vi "SeqEditor_ParamINput.vi"(8 "error in (no error)":errorcluster, 11 "NLTest in":refnum<class "NLTest.lvclass">) -> (0 "error out":errorcluster, 3 "NLTest out":refnum<class "NLTest.lvclass">)   [LabVIEW 2017, in "NLTest.lvclass"]
uses:
  NLTest.lvclass
  NLTest.lvclass/NLTest.ctl
  <vilib>/Utility/miscctls.llb/LVRowAndColumnTypeDef.ctl
  <vilib>/Utility/miscctls.llb/LVSelectionTypeDef.ctl
  SeqEditor_Global.vi
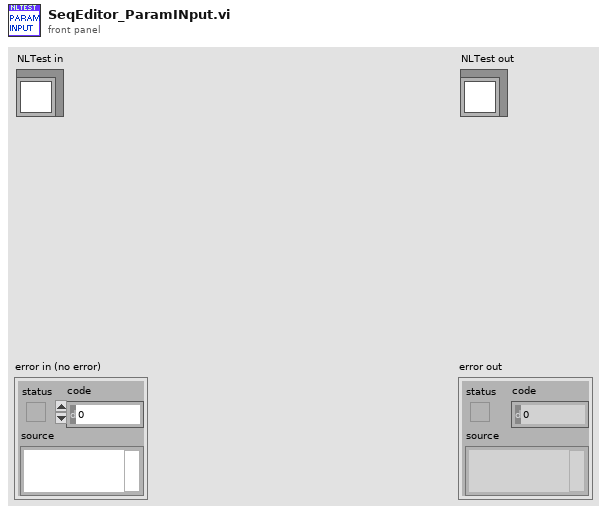
[diagram p1: front panel]
types:
  T1 = typedef "LVRowAndColumnTypeDef.ctl" = cluster{"Row":i32, "Column":i32}
  T2 = typedef "LVSelectionTypeDef.ctl" = cluster{"Selection Start":u32, "Selection End":u32}
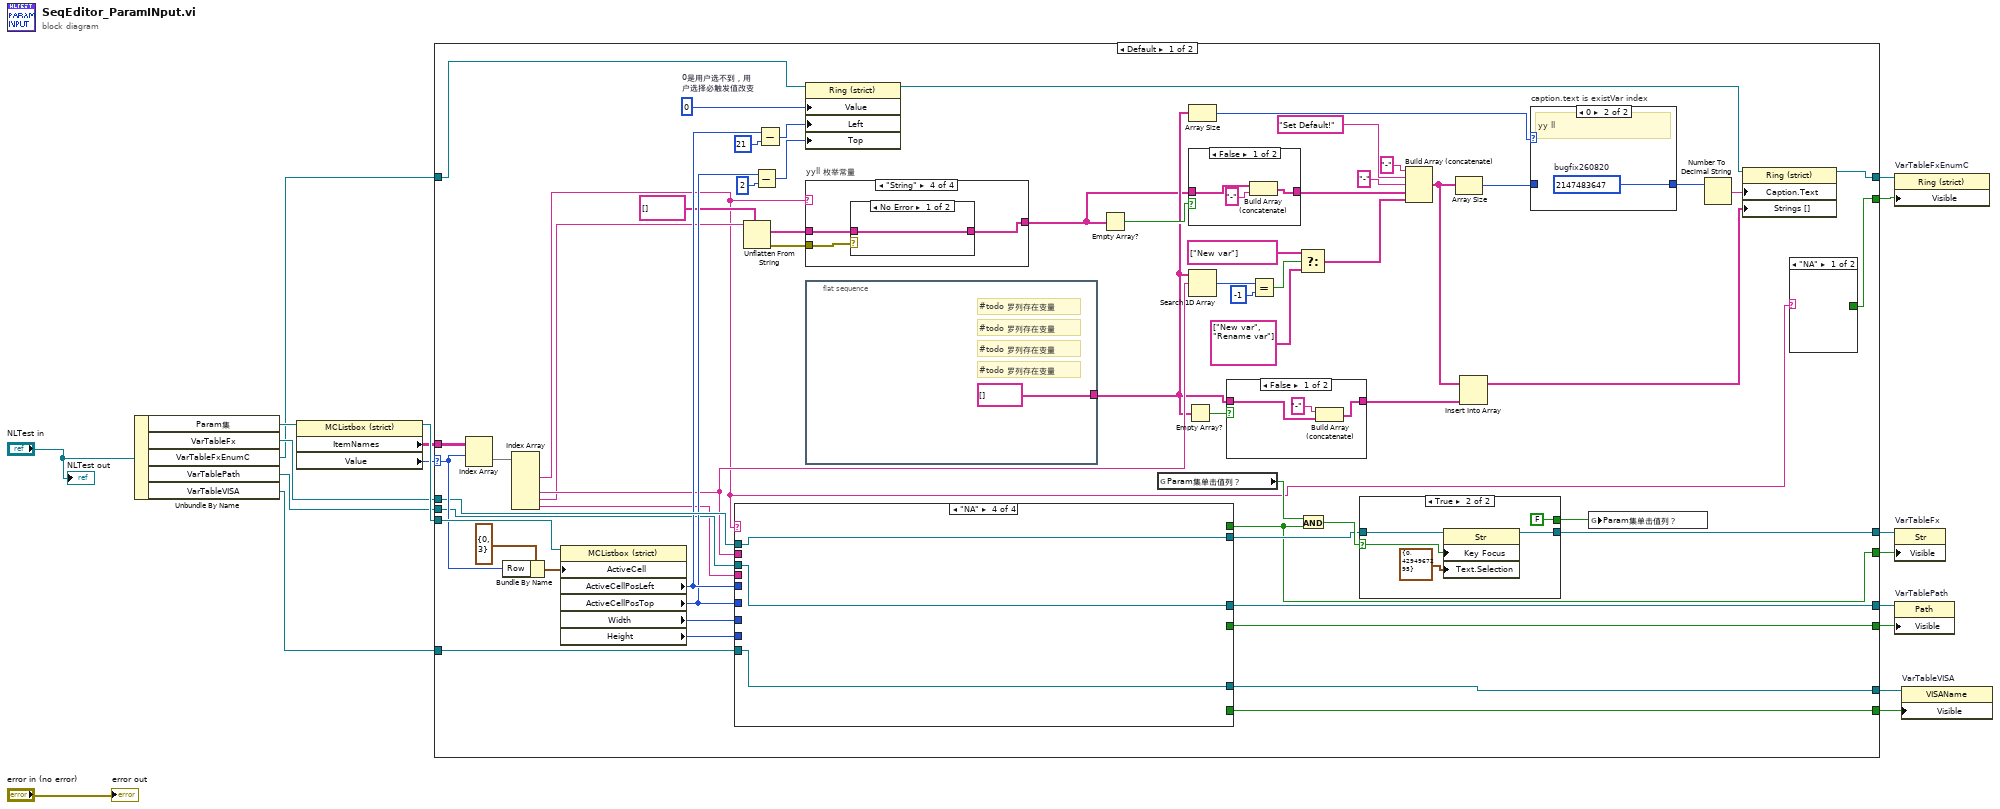
[diagram p0: block diagram]
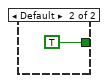
[diagram p2: hidden frame]
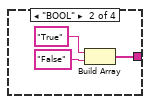
[diagram p4: hidden frame]
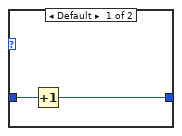
[diagram p7: hidden frame]
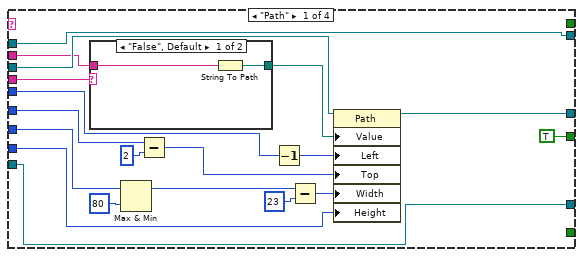
[diagram p11: hidden frame]
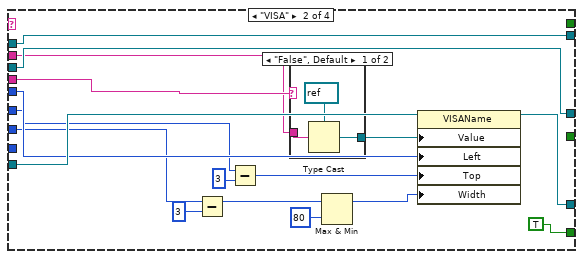
[diagram p13: hidden frame]
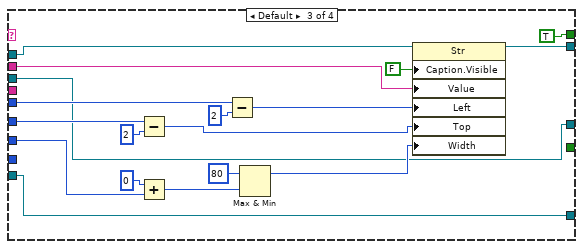
[diagram p15: hidden frame]
diagram:
  n1 = Unbundle By Name("NLTest in") -> ("Param集"=w16:refnum<vi>, "VarTableFx"=w12:refnum<vi>, "VarTableFxEnumC"=w9:refnum<vi>, "VarTablePath"=w5:refnum<vi>, "VarTableVISA"=w1:refnum<vi>)
  n2 = property on="Property Node" class="MCListbox (strict)"(reference=w16) -> (reference out=w15:refnum<vi>, "ItemNames"=w14:string[][], "Value"=w13:i32)  [unwired: 1 in, 1 out]
  n3 = case shown="Default" w13 {
    selector: w13 -> [w74 _]
    tunnel: w15 -> [w78 _]
    tunnel: w14 -> [w77 _]
    tunnel: w12 -> [w72 w170]
    tunnel: [w58 w170] -> w11
    tunnel: [w28 _] -> w10
    tunnel: w9 -> [w68 w171]
    tunnel: [w39 w171] -> w8
    tunnel: [w27 _] -> w7
    tunnel: [w26 _] -> w6
    tunnel: w5 -> [w25 w169]
    tunnel: [w24 w169] -> w4
    tunnel: w1 -> [w22 w168]
    tunnel: [w21 w168] -> w3
    tunnel: [w20 _] -> w2
    frame Default {
      w69 = u16 0  # 0是用户选不到，用 户选择必触发值改变
      n4 = Index Array(array=w77, index (row)=w74) -> (element=w76:string[])  [unwired: 1 in]
      n5 = Bundle By Name(cluster=T1 {"Row"=0, "Column"=3} ("Active Cell:Active Cell"), "Row"=w74) -> (w75:T1)
      n6 = Index Array(array=w76) -> (element #2=w19:string, element #4=w35:string, element #5=w29:string, element #6=w23:string)  [unwired: 6 in, 2 out]
      n7 = property class="MCListbox (strict)"(reference=w78, "ActiveCell"=w75) -> ("ActiveCellPosLeft"=w63:i32, "ActiveCellPosTop"=w62:i32, "Width"=w71:u32, "Height"=w70:u32)  [unwired: 1 in, 2 out]
      n8 = case shown="\"NA\"" w19 {
        tunnel: w72 -> [w124 w134 w157 w167]
        tunnel: w35 -> [w112 w132 w156 _]
        tunnel: w63 -> [w110 w131 w155 _]
        tunnel: w62 -> [w109 w130 w154 _]
        tunnel: w71 -> [w108 w129 w153 _]
        tunnel: w70 -> [w107 _ _ _]
        tunnel: [w124 w134 w151 w167] -> w59
        tunnel: [_ _ TRUE _] -> w27
        tunnel: [TRUE _ _ _] -> w26
        tunnel: w25 -> [w114 w135 w148 w166]
        tunnel: [w113 w135 w148 w166] -> w24
        tunnel: w23 -> [w111 w133 _ _]
        tunnel: w22 -> [w106 w138 w147 w165]
        tunnel: [w106 w137 w147 w165] -> w21
        tunnel: [_ TRUE _ _] -> w20
        frame "Path" {
          n9 = case shown="\"False\", Default" w111 {
            tunnel: w112 -> [w126 _]
            tunnel: [w125 _] -> w122
            frame "False", Default {
              n10 = String To Path(string=w126) -> (path=w125:path)
            }
            frame "True" {
            }
          }
          n11 = Max & Min(x=w108, y=u32 80) -> (max(x,y)=w118:u32)  [unwired: 1 out]
          n12 = Subtract(x=w109, y=2) -> (x-y=w116:i32)
          n13 = Decrement(x=w110) -> (x-1=w117:i32)
          n14 = Subtract(x=w118, y=u32 23) -> (x-y=w121:u32)
          n15 = property class="Path"(reference=w114, "Value"=w122, "Left"=w117, "Top"=w116, "Width"=w121, "Height"=w107) -> (reference out=w113:refnum<vi>)  [unwired: 1 in, 1 out]
        }
        frame "VISA" {
          n16 = Subtract(x=w129, y=u32 3) -> (x-y=w128:u32)
          n17 = Subtract(x=w130, y=3 ("x")) -> (x-y=w140:i32)
          n18 = case shown="\"False\", Default" w133 {
            tunnel: w132 -> [w145 _]
            tunnel: [w144 _] -> w143
            frame "False", Default {
              n19 = Type Cast(type=refnum<visa-resource-name> refnum ("Value"), x=w145) -> (*(type *) &x=w144:refnum<visa-resource-name>)
            }
            frame "True" {
            }
          }
          n20 = Max & Min(x=w128, y=u32 80) -> (max(x,y)=w141:u32)  [unwired: 1 out]
          n21 = property class="VISAName"(reference=w138, "Value"=w143, "Left"=w131, "Top"=w140, "Width"=w141) -> (reference out=w137:refnum<vi>)  [unwired: 1 in, 1 out]
        }
        frame Default {
          n22 = Subtract(x=w154, y=2) -> (x-y=w158:i32)
          n23 = Add(x=u32 0, y=w153) -> (x+y=w162:u32)
          n24 = Subtract(x=w155, y=2 ("x")) -> (x-y=w159:i32)
          n25 = Max & Min(x=u32 80, y=w162) -> (max(x,y)=w161:u32)  [unwired: 1 out]
          n26 = property class="Str"(reference=w157, "Caption.Visible"=FALSE, "Value"=w156, "Left"=w159, "Top"=w158, "Width"=w161) -> (reference out=w151:refnum<vi>)  [unwired: 1 in, 1 out]
        }
        frame "NA" {
        }
      }
      n27 = Unflatten From String(type=string[] [], binary string=w29) -> (value=w32:string[], error out=w31:errorcluster)  [unwired: 3 in, 1 out]
      n28 = Subtract(x=w62, y=2) -> (x-y=w64:i32)
      n29 = Subtract(x=w63, y=21) -> (x-y=w65:i32)
      n30 = property class="Ring (strict)"(reference=w68, "Value"=w69, "Left"=w65, "Top"=w64) -> (reference out=w40:refnum<vi>)  [unwired: 1 in, 1 out]
      n31 = case "yyll 枚举常量" shown="\"String\"" w19 {
        tunnel: w32 -> [w80 _ _ w84]
        tunnel: [w80 w81 _ w85] -> w30
        tunnel: w31 -> [_ _ _ w86]
        frame Default {
        }
        frame "BOOL" {
          n32 = Build Array("True" ("y"), "False" ("y")) -> (w81:string[])
        }
        frame "Number" {
        }
        frame "String" {
          n33 = case shown="No Error" w86 {
            tunnel: [w87 _] -> w85
            tunnel: w84 -> [w87 _]
            frame No Error {
            }
            frame Error {
            }
          }
        }
      }
      n34 = flat-sequence {
        tunnel: [string[] [] ("1D array")] -> w34
        frame #0 {
          # "#todo 罗列存在变量"
          # "#todo 罗列存在变量"
          # "#todo 罗列存在变量"
          # "#todo 罗列存在变量"
        }
      }
      n35 = Empty Array?(array=w30) -> (empty?=w56:bool)
      n36 = global read "SeqEditor_Global.vi" "Param集单击值列？"() -> (w60:bool)
      n37 = Empty Array?(array=w34) -> (empty?=w54:bool)
      n38 = Array Size(array=w34) -> (size(s)=w52:i32)
      n39 = case shown="False" w56 {
        tunnel: [w97 w99] -> w55
        tunnel: w30 -> [w98 w99]
        frame False {
          n40 = Build Array (concatenate)(w98, "-" ("element")) -> (w97:string[])
        }
        frame True {
        }
      }
      n41 = Search 1D Array(1D array=w34, element=w35) -> (index of element=w38:i32)  [unwired: 1 in]
      n42 = case shown="False" w54 {
        tunnel: [w93 w95] -> w53
        tunnel: w34 -> [w94 w95]
        frame False {
          n43 = Build Array (concatenate)("-" ("element"), w94) -> (w93:string[])
        }
        frame True {
        }
      }
      n44 = Equal?(x=w38, y=-1) -> (x = y?=w36:bool)
      n45 = Select(t=string[] ["New var"], s=w36, f=string[] ["New var", "Rename var"]) -> (s? t:f=w44:string[])
      n46 = And(x=w60, y=w27) -> (x .and. y?=w61:bool)
      n47 = case shown="True" w61 {
        selector: w61 -> [_ w103]
        tunnel: [_ FALSE ("Parmcol2hit")] -> w57
        tunnel: w59 -> [w100 w104]
        tunnel: [w100 w101] -> w58
        frame False {
        }
        frame True {
          n48 = property class="Str"(reference=w104, "Key Focus"=w103, "Text.Selection"=T2 {"Selection Start"=0, "Selection End"=4294967295}) -> (reference out=w101:refnum<vi>)  [unwired: 1 in, 1 out]
        }
      }
      n49 = Build Array (concatenate)("-" ("element"), "Set Default!" ("String"), "-" ("element"), w55, w44) -> (w50:string[])
      n50 = Array Size(array=w50) -> (size(s)=w49:i32)
      n51 = Insert Into Array(array=w50, new element=w53) -> (w47:string[])  [unwired: 1 in]
      n52 = case "caption.text is existVar index" shown="0" w52 {
        tunnel: [w89 w91] -> w51
        tunnel: w49 -> [w90 _]
        frame Default {
          n53 = Increment(x=w90) -> (x+1=w89:i32)
        }
        frame 0 {
          w91 = 2147483647  # bugfix260820
          # "yy ll"
        }
      }
      n54 = global write "SeqEditor_Global.vi" "Param集单击值列？"(w57) -> ()
      n55 = Number To Decimal String(number=w51) -> (decimal integer string=w46:string)  [unwired: 1 in]
      n56 = property class="Ring (strict)"(reference=w40, "Caption.Text"=w46, "Strings []"=w47) -> (reference out=w39:refnum<vi>)  [unwired: 1 in, 1 out]
      n57 = case shown="\"NA\"" w19 {
        tunnel: [_ TRUE] -> w28
        frame "NA" {
        }
        frame Default {
        }
      }
    }
    frame ..-1 {
    }
  }
  n58 = property on="VarTableFxEnumC" class="Ring (strict)"(reference=w8, "Visible"=w10) -> ()  [unwired: 1 in, 2 out]
  n59 = property on="VarTableFx" class="Str"(reference=w11, "Visible"=w7) -> ()  [unwired: 1 in, 2 out]
  n60 = property on="VarTablePath" class="Path"(reference=w4, "Visible"=w6) -> ()  [unwired: 1 in, 2 out]
  n61 = property on="VarTableVISA" class="VISAName"(reference=w3, "Visible"=w2) -> ()  [unwired: 1 in, 2 out]
  "error out" <- "error in (no error)"
  "NLTest out" <- "NLTest in"
